vi "serial.vi"() -> ()   [LabVIEW 2017]
uses:
  <vilib>/Instr/_visa.llb/VISA Configure Serial Port (Instr).vi
panel:
  out "SUICHE":bool
  out "TEMPERATURA":dbl(slide) scale=0.0..100.0
  out "read buffer":string
  in  "PUERTO":refnum<visa-resource-name>="COM1"
  in  "POTENCIA":dbl(knob) scale=0.0..100.0
  in  "LED1":bool
  in  "stop":bool
  # "GIRO"
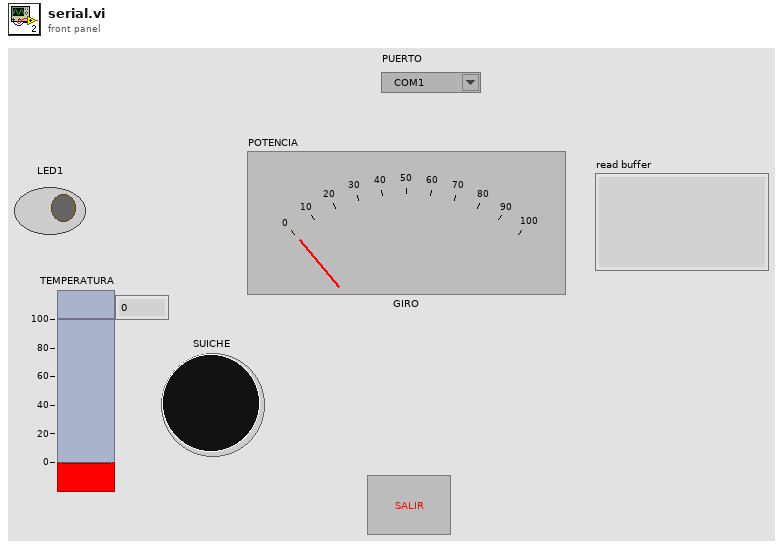
[diagram p1: front panel]
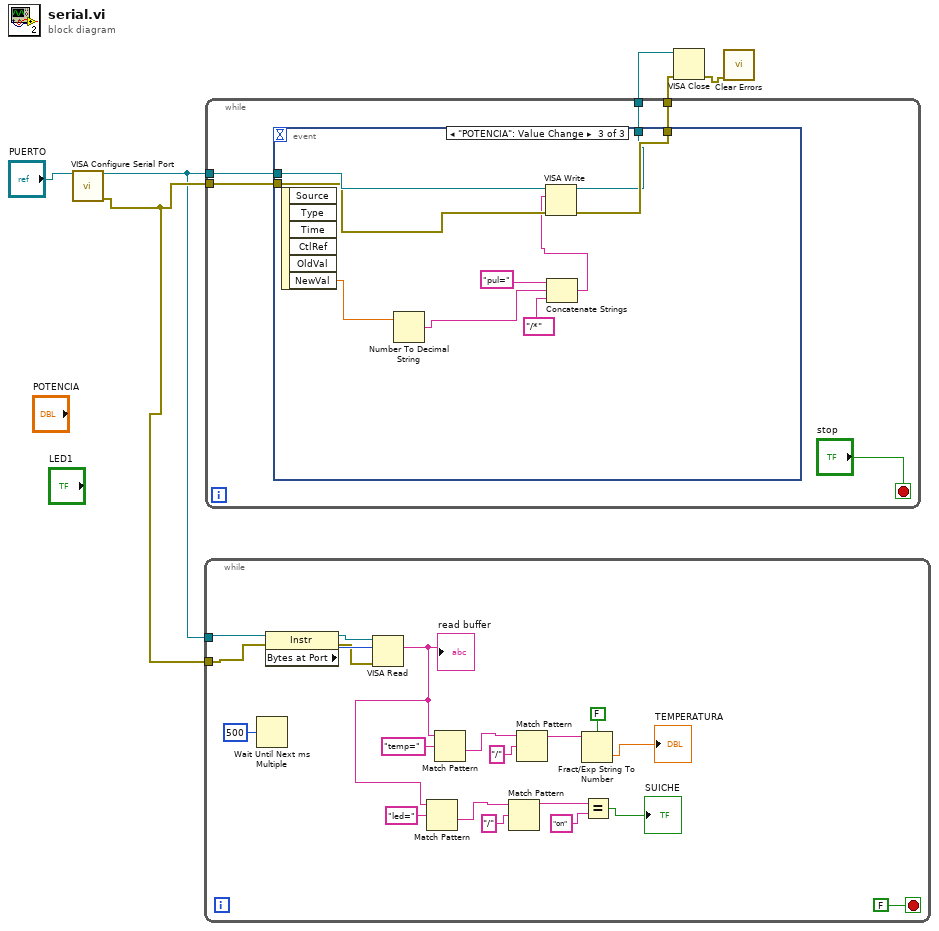
[diagram p0: block diagram]
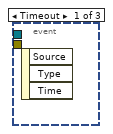
[diagram p2: hidden frame]
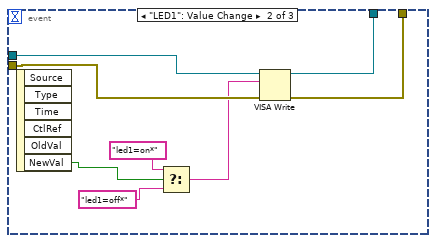
[diagram p3: hidden frame]
diagram:
  n1 = call-poly "VISA Configure Serial Port"("VISA resource name"="PUERTO") -> ("VISA resource name out"=w1:refnum<visa-resource-name>, "error out"=w2:errorcluster)  [unwired: 13 in]
  n2 = while {
    tunnel: w2 -> [w21]
    tunnel: w1 -> [w22]
    stop <- FALSE stop-if-true
    n3 = Wait Until Next ms Multiple(millisecond multiple=u32 500) -> ()  [unwired: 1 out]
    n4 = property class="Instr"(reference=w22, error in=w21) -> (reference out=w24:refnum<visa-resource-name>, error out=w23:errorcluster, "Bytes at Port"=w25:u32)
    n5 = VISA Read(VISA resource name=w24, byte count=w25, error in (no error)=w23) -> (read buffer=w8:string)  [unwired: 3 out]
    "read buffer" <- w8
    n6 = Match Pattern(string=w8, regular expression="led=") -> (after substring=w12:string)  [unwired: 1 in, 3 out]
    n7 = Match Pattern(string=w8, regular expression="temp=") -> (after substring=w18:string)  [unwired: 1 in, 3 out]
    n8 = Match Pattern(string=w12, regular expression="/") -> (before substring=w10:string)  [unwired: 1 in, 3 out]
    n9 = Match Pattern(string=w18, regular expression="/") -> (before substring=w16:string)  [unwired: 1 in, 3 out]
    n10 = Fract/Exp String To Number(use system decimal point (T)=FALSE, string=w16) -> (number=→"TEMPERATURA":dbl)  [unwired: 2 in, 1 out]
    n11 = Equal?(x=w10, y="on") -> (x = y?=→"SUICHE":bool)
  }
  n12 = while {
    tunnel: w1 -> [w30]
    tunnel: w2 -> [w29]
    tunnel: [w28] -> w5
    tunnel: [w27] -> w4
    stop <- "stop" stop-if-true
    n13 = event shown="[2] \"POTENCIA\": Value Change" {
      selector: _ -> [_ _ _]
      dyn-events: _ -> [_ _ _]
      timeout: _ -> [_ _ _]
      tunnel: w30 -> [_ w39 w48]
      tunnel: w29 -> [_ w38 w47]
      tunnel: [_ w33 w45] -> w28
      tunnel: [_ w32 w46] -> w27
      event Timeout {
        n14 = event-data() -> ()  [unwired: 1 in, 3 out]
      }
      event "LED1": Value Change {
        n15 = event-data() -> ("NewVal"=w37:bool)  [unwired: 1 in, 5 out]
        n16 = Select(t="led1=on*", s=w37, f="led1=off*") -> (s? t:f=w34:string)
        n17 = VISA Write(VISA resource name=w39, write buffer=w34, error in (no error)=w38) -> (VISA resource name out=w33:refnum<visa-resource-name>, error out=w32:errorcluster)  [unwired: 1 out]
      }
      event "POTENCIA": Value Change {
        n18 = event-data() -> ("NewVal"=w40:dbl)  [unwired: 1 in, 5 out]
        n19 = Number To Decimal String(number=w40) -> (decimal integer string=w43:string)  [unwired: 1 in]
        n20 = Concatenate Strings("pul=" ("string"), w43, "/*" ("string")) -> (w41:string)
        n21 = VISA Write(VISA resource name=w48, write buffer=w41, error in (no error)=w47) -> (VISA resource name out=w45:refnum<visa-resource-name>, error out=w46:errorcluster)  [unwired: 1 out]
      }
    }
  }
  n22 = VISA Close(VISA resource name=w5, error in (no error)=w4) -> (error out=w3:errorcluster)
  n23 = call <vilib>:"Clear Errors.vi"("error in (no error)"=w3) -> ()  [unwired: 5 in, 2 out]
